vi "ReversedEngineering CreateNodes.vi"(1 "GraphRefToAddNodesTo":refnum<class "Graph.lvclass">, 2 "NodeClassInfoArray":T5[](array[typedef]), 3 "NodeClassInfo":T5, 4 "TypeDefs":T1[](array[typedef]), 5 "error in (no error)":errorcluster, 6 "Show Methods":bool=TRUE, 7 "graphics":refnum<class "Graphics.lvclass">, 8 "Show Attributes":bool=TRUE, 9 "grid":refnum<class "Grid.lvclass">, 11 "CreateTypeDefs":bool) -> (19 "error out":errorcluster)   [LabVIEW 2020]
uses:
  <resource>/Framework/Providers/Open_GDS/UML/ReversedEngineering/ReversedEngineering ClassInfoType.ctl
  <resource>/Framework/Providers/Open_GDS/ClassProviders/Common/CommonVIs/CommonVIs_VisibilityType.ctl
  <resource>/Framework/Providers/Open_GDS/ClassProviders/Common/CommonVIs/CommonVIs_AttributeInfoType.ctl
  <resource>/Framework/Providers/Open_GDS/ClassProviders/Common/CommonVIs/CommonVIs_AttributeDataType.ctl
  <resource>/Framework/Providers/Open_GDS/UML/ReversedEngineering/ReversedEngineering_ClassDependencyDetailsType.ctl
  <resource>/Framework/Providers/Open_GDS/ClassProviders/Common/ScriptingFunctions/SubVIs/Scripting_ViDependencyType.ctl
  <resource>/Framework/Providers/Open_GDS/UML/Graph_class/Graph.lvclass
  <resource>/Framework/Providers/Open_GDS/UML/Graphics_class/Graphics.lvclass
  <resource>/Framework/Providers/Open_GDS/UML/Grid_class/Grid.lvclass
  <resource>/Framework/Providers/Open_GDS/ClassProviders/Common/CommonVIs/CommonVIs_TypeDefType.ctl
  <resource>/Framework/Providers/Open_GDS/UML/ClassNode_class/ExternalSetTypes.ctl
  <resource>/Framework/Providers/Open_GDS/UML/ClassNode_class/ClassNode.lvclass
  C:/Program Files (x86)/National Instruments/LabVIEW 2020/resource/Framework/Providers/Open_GDS/UML/RectangularNode_class/RectangularNode.lvclass
  C:/Program Files (x86)/National Instruments/LabVIEW 2020/resource/Framework/Providers/Open_GDS/UML/AbstractNode_class/AbstractNode.lvclass
  <resource>/Framework/Providers/Open_GDS/UML/InterfaceNode_class/InterfaceNode.lvclass
  C:/Program Files (x86)/National Instruments/LabVIEW 2020/resource/Framework/Providers/Open_GDS/UML/ClassNode_class/ClassNode.lvclass
  <resource>/Framework/Providers/Open_GDS/UML/AbstractNode_class/AbstractNode.lvclass
  <resource>/Framework/Providers/Open_GDS/UML/RectangularNode_class/RectangularNode.lvclass
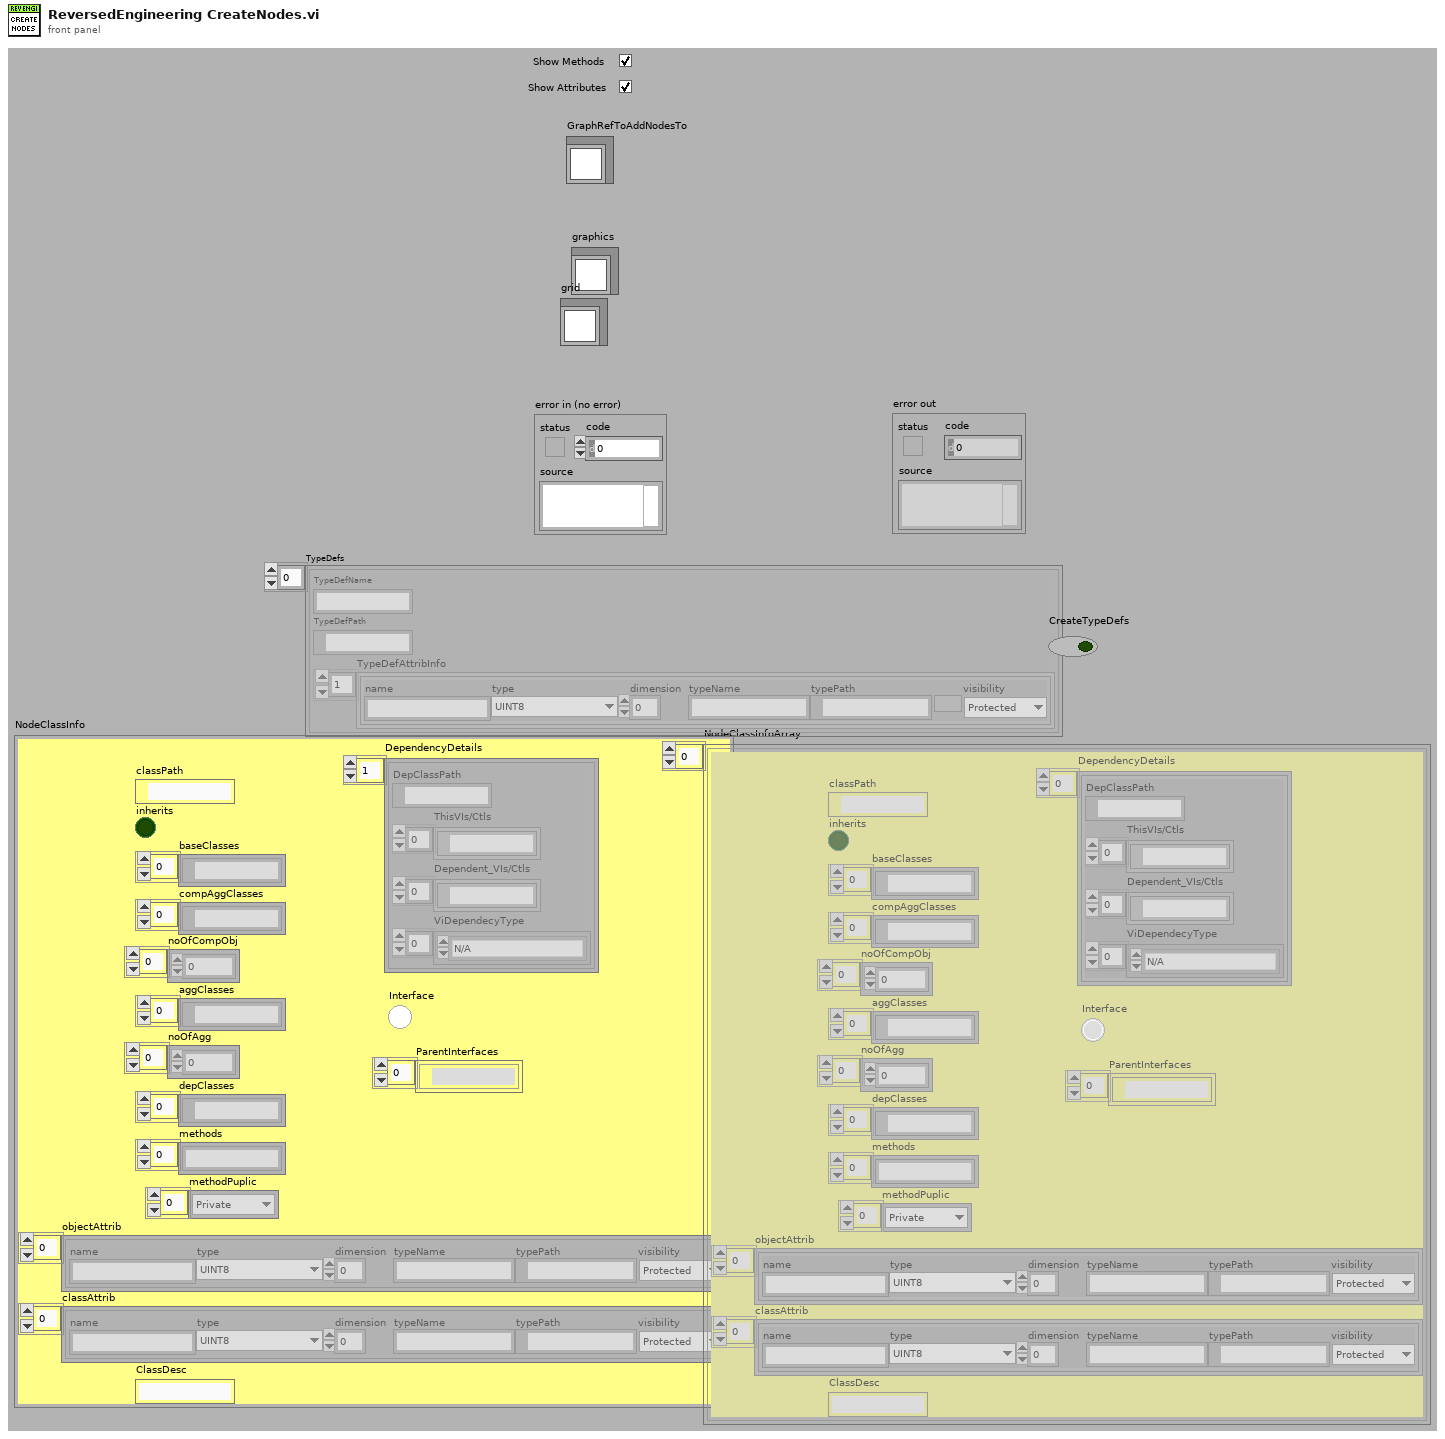
[diagram p1: front panel]
types:
  T1 = typedef "CommonVIs_TypeDefType.ctl" = cluster{"TypeDefName":string, "TypeDefPath":path, "TypeDefAttribInfo":T2[]}
  T2 = typedef "CommonVIs_AttributeInfoType.ctl" = cluster{"name":string, "type":T3, "dimension":i32, "typeName":string, "typePath":path, "visibility":T4}
  T3 = typedef "CommonVIs_AttributeDataType.ctl" = enum16{"UINT8", "INT8", "UINT16", "INT16", "UINT32", "INT32", "UINT64", "INT64", "SGL", "DBL", "EXT", "CSG", "CDB", "CXT", "TimeStamp", "STRING", "PATH", "BOOL", "ENUM", "RefNum", "VIRefNum", "LabVIEW Class", "Cluster", "Variant", "TypeDef", "Waveform", "LabVIEW Object", "Other", "void", "Set", "Map"}
  T4 = typedef "CommonVIs_VisibilityType.ctl" = enum16{"Public", "Private", "Protected"}
  T5 = typedef "ReversedEngineering ClassInfoType.ctl" = cluster{"classPath":path, "inherits":bool, "baseClasses":path[], "compAggClasses":path[], "noOfCompObj":i32[], "aggClasses":path[], "noOfAgg":i32[], "depClasses":path[], "methods":string[], "methodPuplic":T4[], "objectAttrib":T2[], "classAttrib":T2[], "ClassDesc":string, "DependencyDetails":T6[], "Interface":bool, "ParentInterfaces":path[]}
  T6 = typedef "ReversedEngineering_ClassDependencyDetailsType.ctl" = cluster{"DepClassPath":path, "ThisVIs/Ctls":path[], "Dependent_VIs/Ctls":path[], "ViDependecyType":T7[]}
  T7 = typedef "Scripting_ViDependencyType.ctl" = enum16{"N/A", "Launches"}
  T8 = typedef "ClassNode.lvclass/ExternalSetTypes.ctl" = enum16{"Name", "Attributes", "Methods", "Position", "ShowMethods", "ShowAttributes", "ClassPath"}
  T9 = typedef "Rectangle Rectangle2D.ctl" = cluster{"x":dbl, "y":dbl, "width":dbl, "height":dbl}
  T10 = typedef "Point Point2D.ctl" = cluster{"x":dbl, "y":dbl}
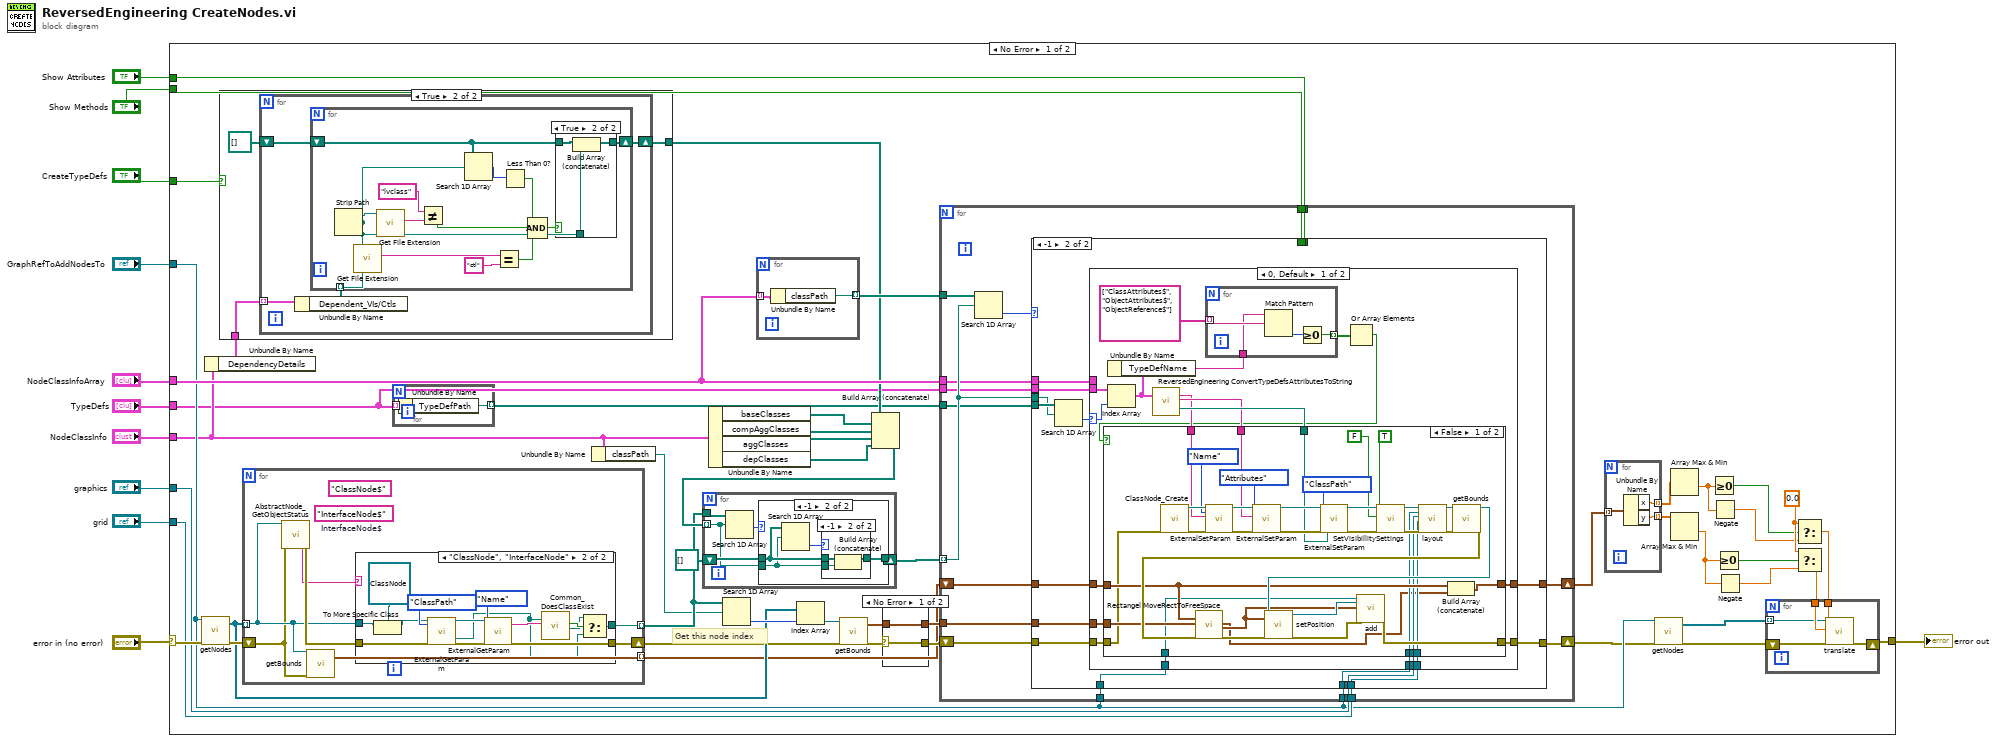
[diagram p0: block diagram]
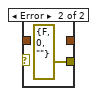
[diagram p4: hidden frame]
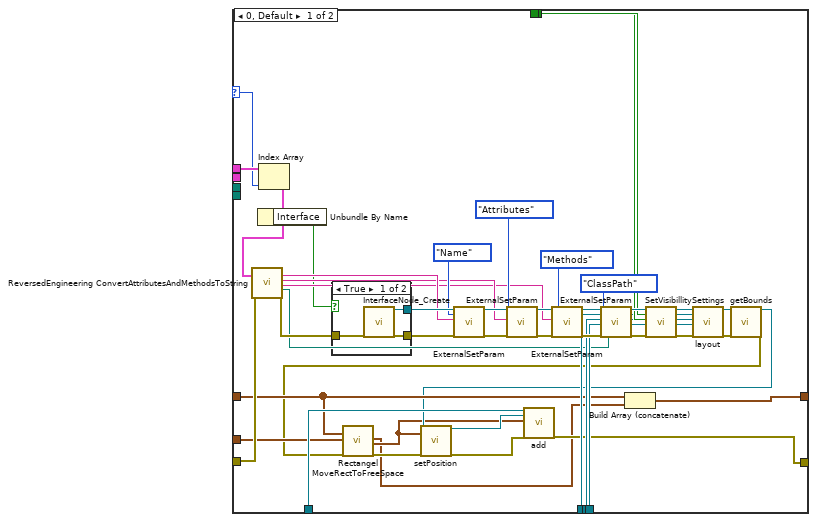
[diagram p7: hidden frame]
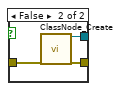
[diagram p8: hidden frame]
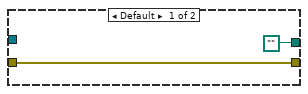
[diagram p11: hidden frame]
diagram:
  n1 = case shown="No Error" "error in (no error)" {
    selector: "error in (no error)" -> [w59 w281]
    tunnel: [w22 w281] -> w10
    tunnel: "Show Methods" -> [w40 _]
    tunnel: "NodeClassInfo" -> [w18 _]
    tunnel: "GraphRefToAddNodesTo" -> [w30 _]
    tunnel: "NodeClassInfoArray" -> [w52 _]
    tunnel: "Show Attributes" -> [w41 _]
    tunnel: "graphics" -> [w39 _]
    tunnel: "grid" -> [w38 _]
    tunnel: "CreateTypeDefs" -> [w14 _]
    tunnel: "TypeDefs" -> [w12 _]
    frame No Error {
      w32 = 0.0 ("t")
      # "Get this node index"
      n2 = call-dynamic "getNodes.vi"("reference"=w30, "error in (no error)"=w59) -> ("nodes"=w47:refnum<class "AbstractNode.lvclass">[], "error out"=w58:errorcluster)  [unwired: 15 in, 1 out]
      n3 = Unbundle By Name(w18) -> ("DependencyDetails"=w17:T6[])
      n4 = case shown="True" w14 {
        tunnel: w17 -> [_ w64]
        tunnel: [_ w63] -> w15
        frame False {
        }
        frame True {
          n5 = for {
            tunnel: w64 -> [w68] mode=indexing
            shift-right: [w66] -> w63
            shift-left: path[] [] -> [w65]
            n6 = Unbundle By Name(w68) -> ("Dependent_VIs/Ctls"=w67:path[])
            n7 = for {
              tunnel: w67 -> [w74] mode=indexing
              shift-right: [w77] -> w66
              shift-left: w65 -> [w76]
              n8 = Strip Path(path=w74) -> (stripped path=w81:path)  [unwired: 1 out]
              n9 = call <vilib>:"Get File Extension.vi"("file"=w74) -> ("lowercase file extension"=w80:string)  [unwired: 1 in, 9 out]
              n10 = call <vilib>:"Get File Extension.vi"("file"=w81) -> ("lowercase file extension"=w72:string)  [unwired: 1 in, 9 out]
              n11 = Not Equal?(x="lvclass", y=w72) -> (x != y?=w69:bool)
              n12 = Search 1D Array(1D array=w76, element=w74) -> (index of element=w75:i32)  [unwired: 1 out]
              n13 = Equal?(x=w80, y="ctl") -> (x = y?=w70:bool)
              n14 = Less Than 0?(x=w75) -> (x < 0?=w73:bool)
              n15 = Compound Arithmetic op=AND(w73, w69, w70) -> (w78:bool)
              n16 = case shown="True" w78 {
                tunnel: [w82 w85] -> w77
                tunnel: w76 -> [w82 w84]
                tunnel: w74 -> [_ w83]
                frame False {
                }
                frame True {
                  n17 = Build Array (concatenate)(w84, w83) -> (w85:path[])
                }
              }
            }
          }
        }
      }
      n18 = for {
        tunnel: w47 -> [w261] mode=indexing
        shift-right: [w264] -> w46
        shift-left: w58 -> [w260]
        tunnel: [w263] -> w50 mode=indexing
        tunnel: [w259] -> w19 mode=indexing
        (unwired) "InterfaceNode$"  # InterfaceNode$
        (unwired) "ClassNode$"
        n19 = call <resource>:"AbstractNode_GetObjectStatus.vi"("reference in"=w261, "error in (no error)"=w260) -> ("Class name"=w258:string, "error out"=w262:errorcluster)  [unwired: 16 out]
        n20 = call-dynamic "getBounds.vi"("reference"=w261, "error in (no error)"=w260) -> ("bounds"=w259:T9)  [unwired: 15 in, 2 out]
        n21 = case shown="\"ClassNode\", \"InterfaceNode\"" w258 {
          tunnel: w261 -> [_ w268]
          tunnel: w262 -> [w266 w275]
          tunnel: [w266 w274] -> w264
          tunnel: [path "" w270] -> w263
          frame Default {
          }
          frame "ClassNode", "InterfaceNode" {
            n22 = To More Specific Class(target class=refnum<class "ClassNode.lvclass"> refnum ("reference"), reference=w268) -> (specific class reference=w267:refnum<class "ClassNode.lvclass">)  [unwired: 1 in, 1 out]
            n23 = call <resource>:"ExternalGetParam.vi"("reference"=w267, "setParameter"=ExternalSetTypes."ClassPath", "error in (no error)"=w275) -> ("reference out"=w279:refnum<class "ClassNode.lvclass">, "Path"=w272:path, "error out"=w278:errorcluster)  [unwired: 14 out]
            n24 = call <resource>:"ExternalGetParam.vi"("reference"=w279, "setParameter"=ExternalSetTypes."Name", "error in (no error)"=w278) -> ("string"=w276:string, "error out"=w274:errorcluster)  [unwired: 15 out]
            n25 = call <resource>:"Common_DoesClassExist.vi"("ClassPath"=w272, "ClassName"=w276) -> ("llb-class"=w273:bool, "llb/LvCLass-Path"=w271:path)  [unwired: 16 out]
            n26 = Select(t=w271, s=w273, f=w272) -> (s? t:f=w270:path)
          }
        }
      }
      n27 = for {
        tunnel: w12 -> [w61] mode=indexing
        tunnel: [w60] -> w13 mode=indexing
        n28 = Unbundle By Name(w61) -> ("TypeDefPath"=w60:path)
      }
      n29 = Unbundle By Name(w18) -> ("classPath"=w49:path)
      n30 = Unbundle By Name(w18) -> ("baseClasses"=w16:path[], "compAggClasses"=w57:path[], "aggClasses"=w56:path[], "depClasses"=w55:path[])
      n31 = Search 1D Array(1D array=w50, element=w49) -> (index of element=w48:i32)  [unwired: 1 out]
      n32 = for {
        tunnel: w52 -> [w112] mode=indexing
        tunnel: [w111] -> w51 mode=indexing
        n33 = Unbundle By Name(w112) -> ("classPath"=w111:path)
      }
      n34 = Index Array(array=w47, index=w48) -> (element=w45:refnum<class "AbstractNode.lvclass">)
      n35 = call-dynamic "getBounds.vi"("reference"=w45, "error in (no error)"=w46) -> ("bounds"=w42:T9, "error out"=w44:errorcluster)  [unwired: 15 in, 1 out]
      n36 = Build Array (concatenate)(w15, w16, w57, w56, w55) -> (w54:path[])
      n37 = for {
        tunnel: w54 -> [w97] mode=indexing
        tunnel: w50 -> [w101]
        shift-right: [w98] -> w53
        shift-left: path[] [] -> [w99]
        n38 = Search 1D Array(1D array=w101, element=w97) -> (index of element=w100:i32)  [unwired: 1 out]
        n39 = case shown="-1" w100 {
          tunnel: w99 -> [w102 w105]
          tunnel: [w102 w106] -> w98
          tunnel: w97 -> [_ w104]
          frame 0, Default {
          }
          frame -1 {
            n40 = Search 1D Array(1D array=w105, element=w104) -> (index of element=w103:i32)  [unwired: 1 out]
            n41 = case shown="-1" w103 {
              tunnel: w105 -> [w107 w110]
              tunnel: [w107 w109] -> w106
              tunnel: w104 -> [_ w108]
              frame 0, Default {
              }
              frame -1 {
                n42 = Build Array (concatenate)(w110, w108) -> (w109:path[])
              }
            }
          }
        }
      }
      n43 = case shown="No Error" w44 {
        selector: w44 -> [w95 _]
        tunnel: [w95 errorcluster {"status"=FALSE, "code"=0, "source"=""} ("error in (no error)")] -> w43
        tunnel: w42 -> [w94 _]
        tunnel: [w94 _] -> w37
        frame No Error {
        }
        frame Error {
        }
      }
      n44 = for {
        tunnel: w51 -> [w129]
        tunnel: w53 -> [w127] mode=indexing
        shift-right: [w118] -> w23
        shift-left: w43 -> [w126]
        tunnel: w52 -> [w125]
        tunnel: w41 -> [w124]
        tunnel: w40 -> [w123]
        tunnel: w30 -> [w122]
        tunnel: w39 -> [w121]
        tunnel: w38 -> [w120]
        tunnel: w30 -> [w119]
        tunnel: w37 -> [w117]
        shift-right: [w115] -> w36
        shift-left: w19 -> [w116]
        tunnel: w13 -> [w114]
        tunnel: w12 -> [w113]
        n45 = Search 1D Array(1D array=w129, element=w127) -> (index of element=w128:i32)  [unwired: 1 out]
        n46 = case shown="-1" w128 {
          selector: w128 -> [w156 _]
          tunnel: w127 -> [_ w193]
          tunnel: w126 -> [w158 w188]
          tunnel: w125 -> [w157 w187]
          tunnel: w124 -> [w149 _]
          tunnel: w123 -> [w148 _]
          tunnel: w122 -> [w147 w184]
          tunnel: w121 -> [w146 w183]
          tunnel: w120 -> [w145 w182]
          tunnel: w117 -> [w140 w186]
          tunnel: w119 -> [w144 w185]
          tunnel: [w143 w189] -> w118
          tunnel: w116 -> [w141 w191]
          tunnel: [w142 w190] -> w115
          tunnel: w114 -> [_ w194]
          tunnel: w113 -> [_ w181]
          frame 0, Default {
            n47 = Index Array(array=w157, index=w156) -> (element=w131:T5)
            n48 = call <resource>:"ReversedEngineering ConvertAttributesAndMethodsToString.vi"("classInfo"=w131, "error in (no error)"=w158) -> ("className"=w169:string, "attributes"=w166:string, "methods"=w162:string, "ClassPath"=w132:path, "error out"=w168:errorcluster)  [unwired: 13 out]
            n49 = Unbundle By Name(w131) -> ("Interface"=w130:bool)
            n50 = case shown="True" w130 {
              tunnel: [w177 w180] -> w174
              tunnel: [w176 w179] -> w173
              tunnel: w168 -> [w175 w178]
              frame True {
                n51 = call <resource>:"InterfaceNode_Create.vi"("error in (no error)"=w175) -> ("reference out"=w177:refnum<class "InterfaceNode.lvclass">, "error out"=w176:errorcluster)  [unwired: 17 in]
              }
              frame False {
                n52 = call <resource>:"ClassNode_Create.vi"("error in (no error)"=w178) -> ("reference out"=w180:refnum<class "ClassNode.lvclass">, "error out"=w179:errorcluster)  [unwired: 1 in, 16 out]
              }
            }
            n53 = call-dynamic "ExternalSetParam.vi"("reference"=w174, "setParameter"=ExternalSetTypes."Name", "string"=w169, "error in (no error)"=w173) -> ("reference out"=w171:refnum<class "ClassNode.lvclass">, "error out"=w170:errorcluster)  [unwired: 14 in]
            n54 = call-dynamic "ExternalSetParam.vi"("reference"=w171, "setParameter"=ExternalSetTypes."Attributes", "string"=w166, "error in (no error)"=w170) -> ("reference out"=w164:refnum<class "ClassNode.lvclass">, "error out"=w165:errorcluster)  [unwired: 14 in]
            n55 = call-dynamic "ExternalSetParam.vi"("reference"=w164, "setParameter"=ExternalSetTypes."Methods", "string"=w162, "error in (no error)"=w165) -> ("reference out"=w160:refnum<class "ClassNode.lvclass">, "error out"=w161:errorcluster)  [unwired: 14 in]
            n56 = call-dynamic "ExternalSetParam.vi"("reference"=w160, "setParameter"=ExternalSetTypes."ClassPath", "error in (no error)"=w161, "ClassPath"=w132) -> ("reference out"=w150:refnum<class "ClassNode.lvclass">, "error out"=w151:errorcluster)  [unwired: 14 in]
            n57 = call <resource>:"SetVisibillitySettings.vi"("reference"=w150, "showAttribute"=w149, "showMethods"=w148, "error in (no error)"=w151) -> ("reference out"=w155:refnum<class "ClassNode.lvclass">, "error out"=w154:errorcluster)  [unwired: 14 out]
            n58 = call-dynamic "layout.vi"("reference"=w155, "graph"=w147, "graphics"=w146, "grid"=w145, "error in (no error)"=w154) -> ("reference out"=w153:refnum<class "ClassNode.lvclass">, "error out"=w152:errorcluster)  [unwired: 13 in]
            n59 = call-dynamic "getBounds.vi"("reference"=w153, "error in (no error)"=w152) -> ("reference out"=w137:refnum<class "ClassNode.lvclass">, "error out"=w139:errorcluster)  [unwired: 15 in, 1 out]
            n60 = call <resource>:"Rectangel MoveRectToFreeSpace.vi"("BoundsArray"=w141, "bounds"=w140, "error in (no error)"=w139) -> ("BoundsOut"=w133:T9, "point"=w135:T10, "error out"=w138:errorcluster)  [unwired: 1 in, 13 out]
            n61 = call <resource>:"setPosition.vi"("reference"=w137, "pos"=w135, "error in (no error)"=w138) -> ("reference out"=w136:refnum<class "ClassNode.lvclass">, "error out"=w134:errorcluster)  [unwired: 2 in, 13 out]
            n62 = call-dynamic "add.vi"("reference"=w144, "node"=w136, "point"=w135, "error in (no error)"=w134) -> ("error out"=w143:errorcluster)  [unwired: 13 in, 2 out]
            n63 = Build Array (concatenate)(w141, w133) -> (w142:T9[])
          }
          frame -1 {
            n64 = Search 1D Array(1D array=w194, element=w193) -> (index of element=w192:i32)  [unwired: 1 out]
            n65 = case shown="0, Default" w192 {
              selector: w192 -> [w213 _]
              tunnel: w191 -> [w211 w257]
              tunnel: [w210 w257] -> w190
              tunnel: [w209 w256] -> w189
              tunnel: w188 -> [w203 w256]
              tunnel: w187 -> [_ _]
              tunnel: w186 -> [w212 _]
              tunnel: w185 -> [w208 _]
              tunnel: w184 -> [w207 _]
              tunnel: w183 -> [w206 _]
              tunnel: w182 -> [w205 _]
              tunnel: w181 -> [w204 _]
              frame 0, Default {
                n66 = Index Array(array=w204, index=w213) -> (element=w197:T1)
                n67 = Unbundle By Name(w197) -> ("TypeDefName"=w196:string)
                n68 = call <resource>:"ReversedEngineering ConvertTypeDefsAttributesToString.vi"("TypeDef"=w197) -> ("className"=w200:string, "attributes"=w201:string, "ClassPath"=w202:path)  [unwired: 1 in, 15 out]
                n69 = for {
                  tunnel: [w254] -> w199 mode=indexing
                  tunnel: string[] ["ClassAttributes$", "ObjectAttributes$", "ObjectReference$"] -> [w253] mode=indexing
                  tunnel: w196 -> [w252]
                  n70 = Match Pattern(string=w252, regular expression=w253) -> (offset past match=w255:i32)  [unwired: 4 out]
                  n71 = Greater Or Equal To 0?(x=w255) -> (x >= 0?=w254:bool)
                }
                n72 = Or Array Elements(Boolean array=w199) -> (logical OR=w195:bool)
                n73 = case shown="False" w195 {
                  tunnel: w212 -> [w230 _]
                  tunnel: w211 -> [w229 w251]
                  tunnel: [w228 w251] -> w210
                  tunnel: [w227 w250] -> w209
                  tunnel: w208 -> [w226 _]
                  tunnel: w207 -> [w225 _]
                  tunnel: w206 -> [w224 _]
                  tunnel: w205 -> [w223 _]
                  tunnel: w203 -> [w218 w250]
                  tunnel: w202 -> [w217 _]
                  tunnel: w201 -> [w216 _]
                  tunnel: w200 -> [w215 _]
                  frame False {
                    n74 = call <resource>:"ClassNode_Create.vi"("error in (no error)"=w218) -> ("reference out"=w249:refnum<class "ClassNode.lvclass">, "error out"=w248:errorcluster)  [unwired: 1 in, 16 out]
                    n75 = call-dynamic "ExternalSetParam.vi"("reference"=w249, "setParameter"=ExternalSetTypes."Name", "string"=w215, "error in (no error)"=w248) -> ("reference out"=w246:refnum<class "ClassNode.lvclass">, "error out"=w245:errorcluster)  [unwired: 14 in]
                    n76 = call-dynamic "ExternalSetParam.vi"("reference"=w246, "setParameter"=ExternalSetTypes."Attributes", "string"=w216, "error in (no error)"=w245) -> ("reference out"=w221:refnum<class "ClassNode.lvclass">, "error out"=w222:errorcluster)  [unwired: 14 in]
                    n77 = call-dynamic "ExternalSetParam.vi"("reference"=w221, "setParameter"=ExternalSetTypes."ClassPath", "error in (no error)"=w222, "ClassPath"=w217) -> ("reference out"=w237:refnum<class "ClassNode.lvclass">, "error out"=w238:errorcluster)  [unwired: 14 in]
                    n78 = call <resource>:"SetVisibillitySettings.vi"("reference"=w237, "showAttribute"=TRUE, "showMethods"=FALSE, "error in (no error)"=w238) -> ("reference out"=w242:refnum<class "ClassNode.lvclass">, "error out"=w241:errorcluster)  [unwired: 14 out]
                    n79 = call-dynamic "layout.vi"("reference"=w242, "graph"=w225, "graphics"=w224, "grid"=w223, "error in (no error)"=w241) -> ("reference out"=w240:refnum<class "ClassNode.lvclass">, "error out"=w239:errorcluster)  [unwired: 13 in]
                    n80 = call-dynamic "getBounds.vi"("reference"=w240, "error in (no error)"=w239) -> ("reference out"=w234:refnum<class "ClassNode.lvclass">, "error out"=w236:errorcluster)  [unwired: 15 in, 1 out]
                    n81 = call <resource>:"Rectangel MoveRectToFreeSpace.vi"("BoundsArray"=w229, "bounds"=w230, "error in (no error)"=w236) -> ("BoundsOut"=w214:T9, "point"=w232:T10, "error out"=w235:errorcluster)  [unwired: 1 in, 13 out]
                    n82 = call <resource>:"setPosition.vi"("reference"=w234, "pos"=w232, "error in (no error)"=w235) -> ("reference out"=w233:refnum<class "ClassNode.lvclass">, "error out"=w231:errorcluster)  [unwired: 2 in, 13 out]
                    n83 = call-dynamic "add.vi"("reference"=w226, "node"=w233, "point"=w232, "error in (no error)"=w231) -> ("error out"=w227:errorcluster)  [unwired: 13 in, 2 out]
                    n84 = Build Array (concatenate)(w229, w214) -> (w228:T9[])
                  }
                  frame True {
                  }
                }
              }
              frame -1 {
              }
            }
          }
        }
      }
      n85 = for {
        tunnel: w36 -> [w93] mode=indexing
        tunnel: [w92] -> w35 mode=indexing
        tunnel: [w91] -> w34 mode=indexing
        n86 = Unbundle By Name(w93) -> ("x"=w92:dbl, "y"=w91:dbl)
      }
      n87 = call-dynamic "getNodes.vi"("reference"=w30, "error in (no error)"=w23) -> ("nodes"=w21:refnum<class "AbstractNode.lvclass">[])  [unwired: 15 in, 2 out]
      n88 = Array Max & Min(array=w35) -> (min value=w28:dbl)  [unwired: 3 out]
      n89 = Array Max & Min(array=w34) -> (min value=w26:dbl)  [unwired: 3 out]
      n90 = Greater Or Equal To 0?(x=w28) -> (x >= 0?=w29:bool)
      n91 = Negate(x=w28) -> (-x=w27:dbl)
      n92 = Greater Or Equal To 0?(x=w26) -> (x >= 0?=w25:bool)
      n93 = Negate(x=w26) -> (-x=w24:dbl)
      n94 = Select(t=w32, s=w29, f=w27) -> (s? t:f=w33:dbl)
      n95 = Select(t=w32, s=w25, f=w24) -> (s? t:f=w31:dbl)
      n96 = for {
        tunnel: w33 -> [w90]
        tunnel: w31 -> [w89]
        shift-right: [w87] -> w22
        shift-left: w23 -> [w88]
        tunnel: w21 -> [w86] mode=indexing
        n97 = call-dynamic "translate.vi"("reference"=w86, "dx"=w90, "dy"=w89, "error in (no error)"=w88) -> ("error out"=w87:errorcluster)  [unwired: 14 in, 1 out]
      }
    }
    frame Error {
    }
  }
  "error out" <- w10
